vi "Event GUI QMH Template.vi"   [LabVIEW 2020, in "Volatus.lvlib"]
uses:
  Volatus.lvlib
  Module/Module.lvclass
  MessageQ/MessageQ.lvclass
types:
  T1 = enum32{"Invalid", "Standard", "Closed", "Hidden", "Minimized", "Maximized"}
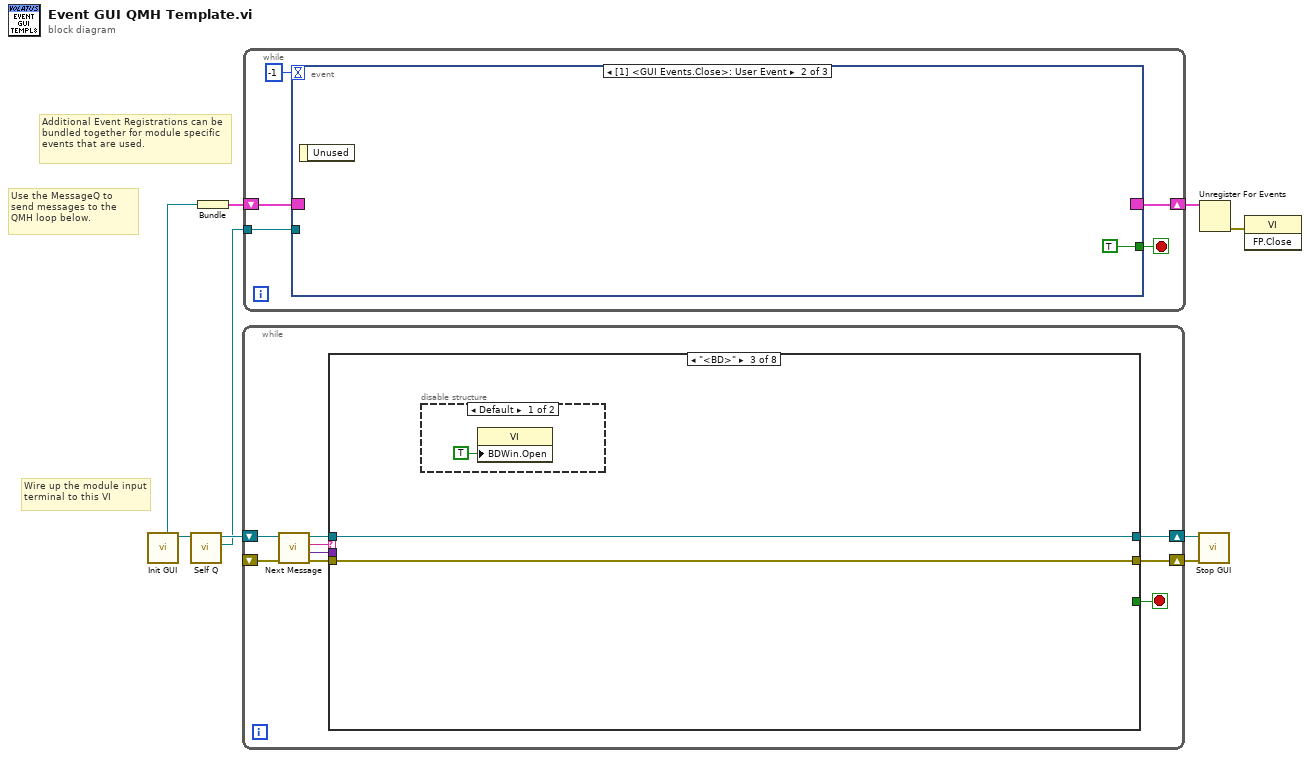
[diagram p0: block diagram]
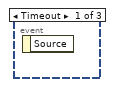
[diagram p2: hidden frame]
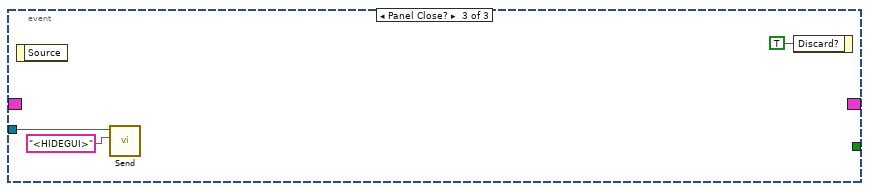
[diagram p3: hidden frame]
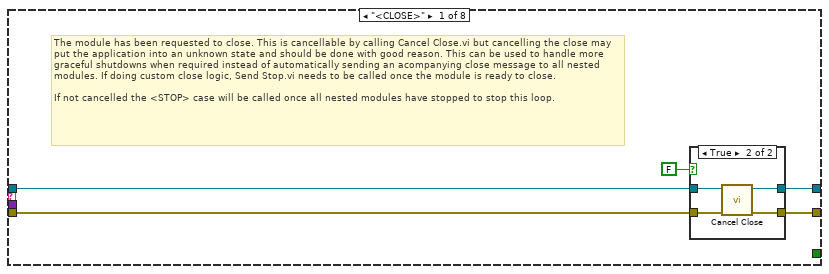
[diagram p4: hidden frame]
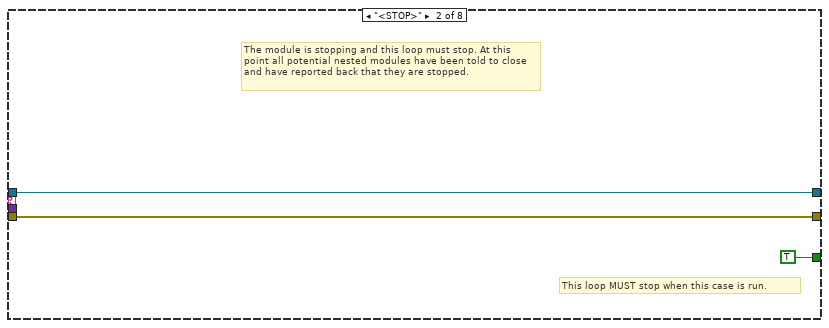
[diagram p6: hidden frame]
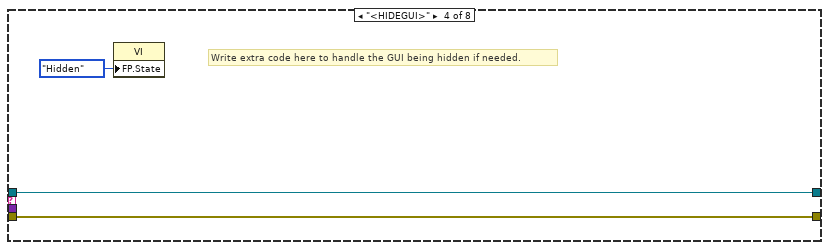
[diagram p8: hidden frame]
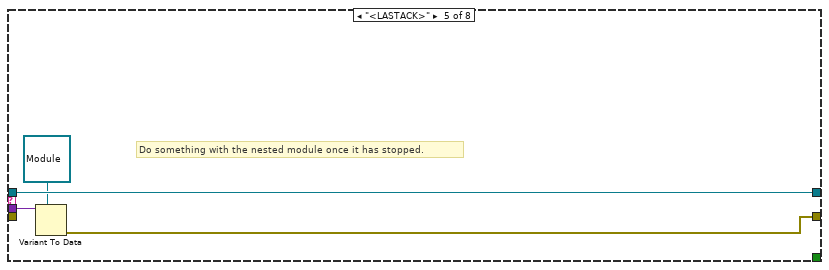
[diagram p9: hidden frame]
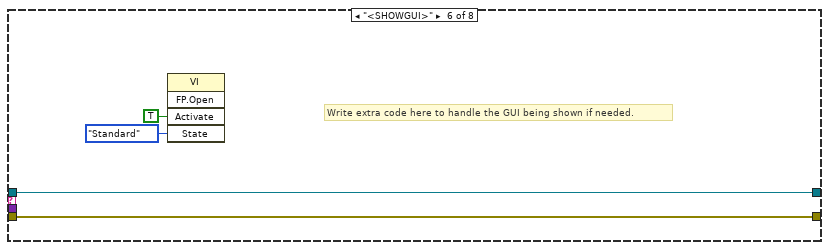
[diagram p10: hidden frame]
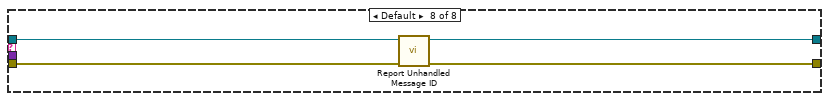
[diagram p12: hidden frame]
diagram:
  # "Additional Event Registrations can be bundled together for module specific events that are used."
  # "Use the MessageQ to send messages to the QMH loop below."
  # "Wire up the module input terminal to this VI"
  n1 = call "Init GUI.vi"() -> ("Module out"=w7:refnum<class "Module.lvclass">, "Event Reg"=w2:refnum<event-registration>)  [unwired: 10 in]
  n2 = call "Self Q.vi"("Module in"=w7) -> ("Self Q"=w8:refnum<class "MessageQ.lvclass">, "Module out"=w9:refnum<class "Module.lvclass">)  [unwired: 9 in]
  n3 = Bundle("Event Reg"=w2) -> (w6:cluster{"Event Reg":refnum<event-registration>})  [unwired: 1 in]
  n4 = while {
    shift-right: [w13] -> w4
    shift-left: w9 -> [w18]
    shift-right: [w12] -> w3
    shift-left: _ -> [w17]
    stop <- w11 stop-if-true
    n5 = call "Next Message.vi"("error in (no error)"=w17, "Module in"=w18) -> ("error out"=w16:errorcluster, "Data"=w10:variant, "ID"=w15:string, "Module out"=w14:refnum<class "Module.lvclass">)  [unwired: 6 in]
    n6 = case shown="\"<BD>\"" w15 {
      tunnel: w16 -> [w21 w31 w33 w37 _ w45 w47 w52]
      tunnel: w14 -> [w22 w32 w34 w38 w42 w46 w48 w50]
      tunnel: [w20 w32 w34 w38 w42 w46 w48 w49] -> w13
      tunnel: [w19 w31 w33 w37 w39 w45 w47 w51] -> w12
      tunnel: [_ TRUE _ _ _ _ _ _] -> w11
      tunnel: w10 -> [_ _ _ _ w41 _ _ _]
      frame "<CLOSE>" {
        # "The module has been requested to close. This is cancellable by calling Cancel Close.vi but cancelling the close may put the application into an unknown state and should be done with good reason. This can be used to handle more graceful shutdowns when required instead of automatically sending an acompanying close message to all nested modules. If doing custom close logic, Send Stop.vi needs to be called once the module is ready to close.\n\nIf not cancelled the <STOP> case will be called once all nested modules have stopped to stop this loop."
        n7 = case shown="True" FALSE {
          tunnel: w21 -> [w24 w29]
          tunnel: [w24 w28] -> w19
          tunnel: w22 -> [w25 w27]
          tunnel: [w25 w26] -> w20
          frame False {
          }
          frame True {
            n8 = call "Cancel Close.vi"("error in (no error)"=w29, "Module in"=w27) -> ("error out"=w28:errorcluster, "Module out"=w26:refnum<class "Module.lvclass">)  [unwired: 8 in]
          }
        }
      }
      frame "<STOP>" {
        # "This loop MUST stop when this case is run."
        # "The module is stopping and this loop must stop. At this point all potential nested modules have been told to close and have reported back that they are stopped."
      }
      frame "<BD>" {
        n9 = disable-structure shown="Default" {
          frame condition #0 (active) {
            n10 = property class="VI"("BDWin.Open"=TRUE ("Block Diagram Window:Open")) -> ()  [unwired: 2 in, 2 out]
          }
          frame condition #1 {
          }
        }
      }
      frame "<HIDEGUI>" {
        # "Write extra code here to handle the GUI being hidden if needed."
        n11 = property class="VI"("FP.State"=T1."Hidden" ("Front Panel Window:State")) -> ()  [unwired: 2 in, 2 out]
      }
      frame "<LASTACK>" {
        # "Do something with the nested module once it has stopped."
        n12 = Variant To Data(type=refnum<class "Module.lvclass"> refnum ("Volatus:Module"), Variant=w41) -> (error out=w39:errorcluster)  [unwired: 1 in, 1 out]
      }
      frame "<SHOWGUI>" {
        # "Write extra code here to handle the GUI being shown if needed."
        n13 = invoke class="VI" method="FP.Open"("Activate"=TRUE ("Activate?"), "State"=T1."Standard") -> ()  [unwired: 3 in, 5 out]
      }
      frame "<TIMEOUT>" {
        # "No message for this module was received in time"
      }
      frame Default {
        n14 = call "Report Unhandled Message ID.vi"("error in (no error)"=w52, "Module in"=w50) -> ("error out"=w51:errorcluster, "Module out"=w49:refnum<class "Module.lvclass">)  [unwired: 8 in]
      }
    }
  }
  n15 = while {
    tunnel: w8 -> [w57]
    shift-right: [w55] -> w5
    shift-left: w6 -> [w56]
    stop <- w54 stop-if-true
    n16 = event shown="[1] <GUI Events.Close>: User Event" {
      selector: w56 -> [_ _ _]
      dyn-events: [_ _ _] -> w55
      timeout: -1 -> [_ _ _]
      tunnel: w57 -> [_ _ w60]
      tunnel: [_ TRUE _] -> w54
      event Timeout {
        n17 = event-data() -> ()  [unwired: 1 in, 1 out]
      }
      event User Event {
        n18 = event-data() -> ()  [unwired: 1 in, 1 out]
      }
      event Panel Close? {
        n19 = event-data() -> ()  [unwired: 1 in, 1 out]
        n20 = call "Send.vi"("ID"="<HIDEGUI>", "MessageQ in"=w60) -> ()  [unwired: 8 in, 2 out]
        n21 = event-data("Discard?"=TRUE) -> ()  [unwired: 1 in, 1 out]
      }
    }
  }
  n22 = call "Stop GUI.vi"("error in (no error)"=w3, "Module in"=w4) -> ()  [unwired: 8 in, 2 out]
  n23 = Unregister For Events(event registration refnum=w5) -> (error out=w1:errorcluster)  [unwired: 1 in]
  n24 = invoke class="VI" method="FP.Close"(error in=w1) -> ()  [unwired: 2 in, 3 out]
